vi "Create Keywords List File from CHM Project.vi"(8 "error in":errorcluster, 11 "HHP file":path) -> (0 "error out":errorcluster, 1 "Keywords List":string, 2 "# keywords":i32, 3 "Output file path":path, 5 ".hhk file":path)   [LabVIEW 2021]
doc: "::: CalcExpress Toolkit :::\nCopyright (c) 2000-2026 Konstantin Shifershteyn. All rights reserved."
uses:
  <vilib>/Utility/config.llb/Read Key (Path).vi
  <vilib>/Utility/config.llb/NI_LVConfig.lvlib
panel:
  # "CalcExpress Toolkit\nCopyright (c) 2000-2026 Konstantin Shifershteyn"
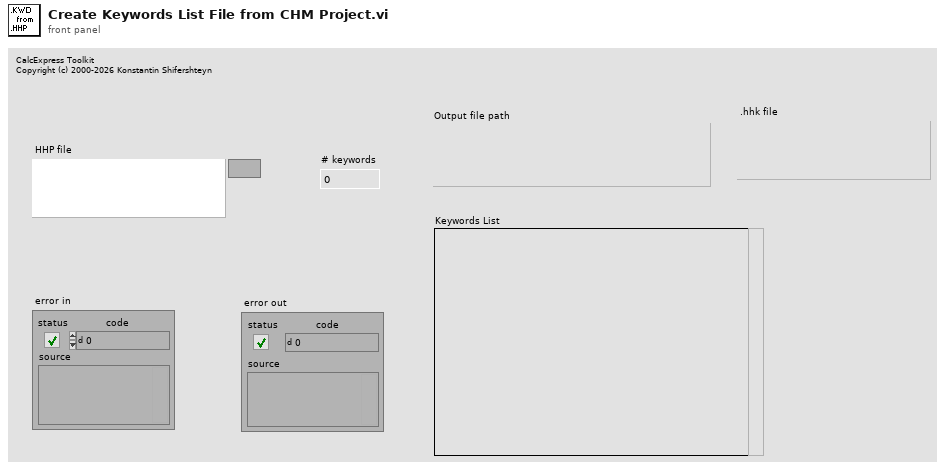
[diagram p1: front panel]
types:
  T1 = typedef "NI_LVConfig.lvlib/Config Data RefNum.ctl" = refnum<k1>
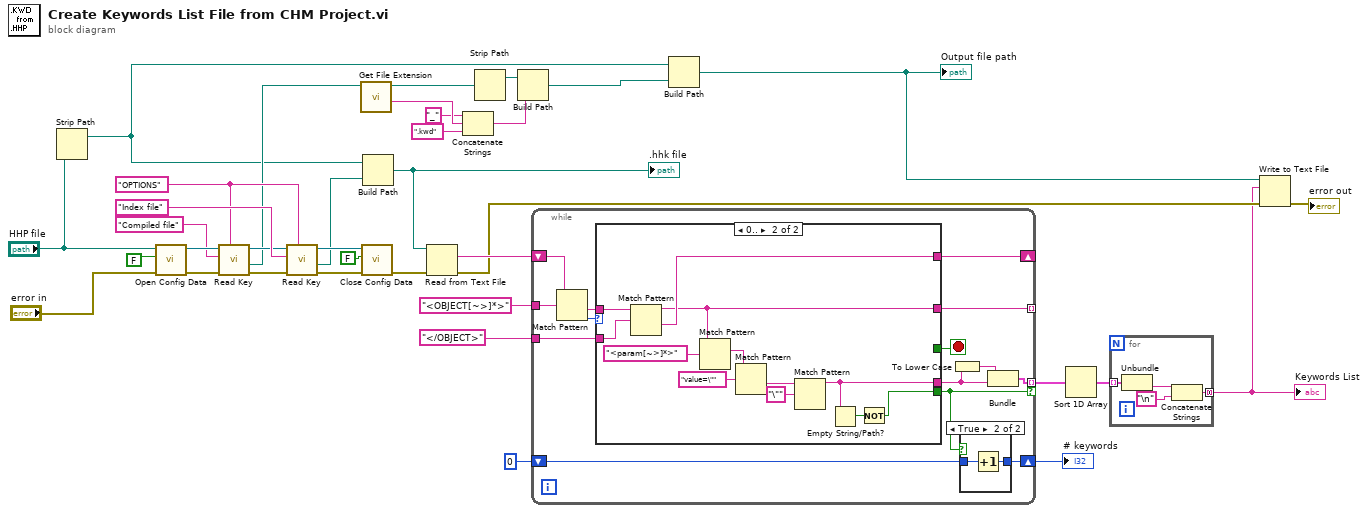
[diagram p0: block diagram]
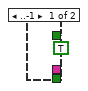
[diagram p3: hidden frame]
diagram:
  w28 = "OPTIONS"
  n1 = Strip Path(path="HHP file") -> (stripped path=w12:path)  [unwired: 1 out]
  n2 = call <vilib>:"Open Config Data.vi"("error in (no error)"="error in", "create file if necessary (T)"=FALSE, "configuration file path"="HHP file") -> ("error out"=w27:errorcluster, "refnum"=w32:T1)  [unwired: 6 in, 1 out]
  n3 = call-poly <vilib>:"Read Key.vi"("section"=w28, "error in (no error)"=w27, "key"="Compiled file", "refnum"=w32) -> ("error out"=w26:errorcluster, "value"=w20:path, "refnum out"=w29:T1)  [unwired: 4 in, 1 out]
  n4 = call-poly <vilib>:"Read Key.vi"("section"=w28, "error in (no error)"=w26, "key"="Index file", "refnum"=w29) -> ("error out"=w24:errorcluster, "value"=w22:path, "refnum out"=w25:T1)  [unwired: 4 in, 1 out]
  n5 = call <vilib>:"Get File Extension.vi"("file"=w20) -> ("filename without extension"=w19:string, "dup file"=w16:path)  [unwired: 6 in, 3 out]
  n6 = call <vilib>:"Close Config Data.vi"("error in (no error)"=w24, "write file if changed (T)"=FALSE, "refnum"=w25) -> ("error out"=w11:errorcluster)  [unwired: 7 in, 1 out]
  n7 = Build Path(base path=w12, name or relative path=w22) -> (appended path=w21:path)
  ".hhk file" <- w21
  n8 = Read from Text File(file (use dialog)=w21, error in=w11) -> (text=w36:string, error out=w10:errorcluster)  [unwired: 2 in, 2 out]
  n9 = Concatenate Strings("_" ("string"), w19, ".kwd" ("string")) -> (w14:string)
  n10 = Strip Path(path=w16) -> (stripped path=w15:path)  [unwired: 1 out]
  n11 = Build Path(base path=w15, name or relative path=w14) -> (appended path=w13:path)
  n12 = while {
    shift-right: [w46] -> _
    shift-left: w36 -> [w50]
    tunnel: "<OBJECT[~>]*>" -> [w49]
    tunnel: "</OBJECT>" -> [w47]
    tunnel: [w45] -> _ mode=indexing
    tunnel: [w39] -> w4 mode=indexing if=w40
    shift-right: [w41] -> w5
    shift-left: 0 -> [w42]
    stop <- w43 stop-if-true
    n13 = Match Pattern(string=w50, regular expression=w49) -> (after substring=w48:string, offset past match=w44:i32)  [unwired: 1 in, 2 out]
    n14 = case shown="0.." w44 {
      tunnel: w48 -> [_ w66]
      tunnel: w47 -> [_ w65]
      tunnel: [_ w64] -> w46
      tunnel: [_ w63] -> w45
      tunnel: [TRUE _] -> w43
      tunnel: [_ w55] -> w38
      tunnel: [_ w57] -> w40
      frame ..-1 {
      }
      frame 0.. {
        n15 = Match Pattern(string=w66, regular expression=w65) -> (before substring=w63:string, after substring=w64:string)  [unwired: 1 in, 2 out]
        n16 = Match Pattern(string=w63, regular expression="<param[~>]*>") -> (match substring=w56:string)  [unwired: 1 in, 3 out]
        n17 = Match Pattern(string=w56, regular expression="value=\"") -> (after substring=w60:string)  [unwired: 1 in, 3 out]
        n18 = Match Pattern(string=w60, regular expression="\"") -> (before substring=w55:string)  [unwired: 1 in, 3 out]
        n19 = Empty String/Path?(string/path=w55) -> (empty?=w58:bool)
        n20 = Not(x=w58) -> (.not. x?=w57:bool)
      }
    }
    n21 = To Lower Case(string=w38) -> (all lower case string=w37:string)
    n22 = case shown="True" w40 {
      tunnel: w42 -> [w51 w53]
      tunnel: [w51 w52] -> w41
      frame False {
      }
      frame True {
        n23 = Increment(x=w53) -> (x+1=w52:i32)
      }
    }
    n24 = Bundle(w37, w38) -> (w39:cluster{string, string})  [unwired: 1 in]
  }
  "# keywords" <- w5
  n25 = Build Path(base path=w12, name or relative path=w13) -> (appended path=w9:path)
  "Output file path" <- w9
  n26 = Sort 1D Array(array=w4) -> (sorted array=w3:cluster{string, string}[])
  n27 = for {
    tunnel: w3 -> [w70] mode=indexing
    tunnel: [w67] -> w2 mode=concatenating
    n28 = Unbundle(w70) -> (w68:string)  [unwired: 1 out]
    n29 = Concatenate Strings(w68, "\n") -> (w67:string)
  }
  "Keywords List" <- w2
  n30 = Write to Text File(file (use dialog)=w9, text=w2, error in=w10) -> (error out=→"error out":errorcluster)  [unwired: 1 in, 2 out]
